vi "Set Channel - GPIO DO.vi"(6 "GPIO Pull":T1, 8 "error in (no error)":errorcluster, 9 "GPIO Number":T2=-1, 10 "Tag":string, 11 "CTI_GPIO_DigitalOut in":refnum<class "CTI_GPIO_DigitalOut.lvclass">) -> (0 "error out":errorcluster, 3 "CTI_GPIO_DigitalOut out":refnum<class "CTI_GPIO_DigitalOut.lvclass">)   [LabVIEW 2021, in "CTI_GPIO_DigitalOut.lvclass"]
uses:
  CTI_GPIO_DigitalOut.lvclass
  <vilib>/CTI/CTI Drivers/CTI/GPIO Number.ctl
  <vilib>/CTI/CTI Drivers/CTI/GPIO Pull.ctl
  <vilib>/CTI/CTI Drivers/CTI/CTI.lvlib
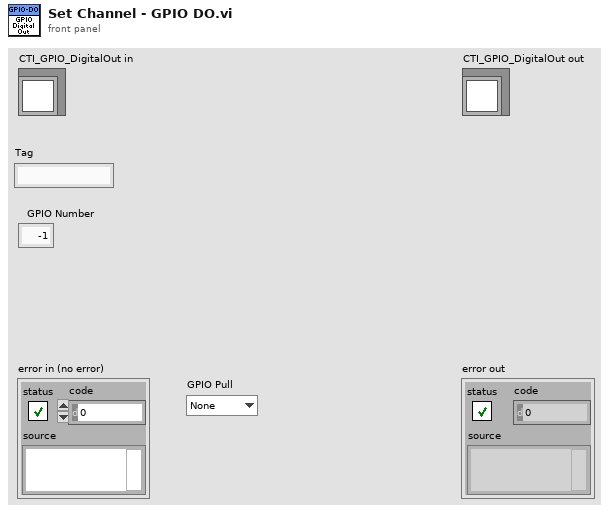
[diagram p1: front panel]
types:
  T1 = typedef "CTI.lvlib/GPIO Pull.ctl" = enum16{"None", "Up", "Down", "Both"}
  T2 = typedef "CTI.lvlib/GPIO Number.ctl" = i8
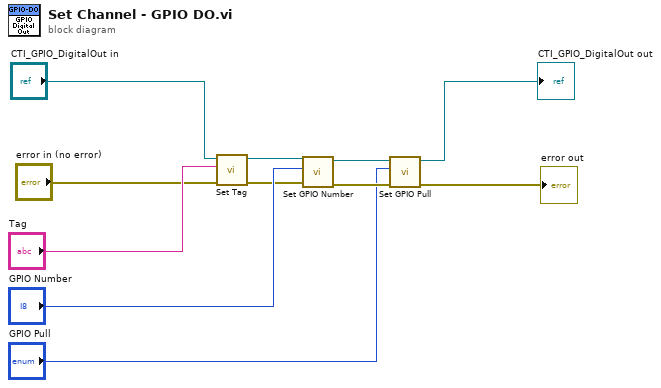
[diagram p0: block diagram]
diagram:
  n1 = call-dynamic "Set Tag.vi"("error in (no error)"="error in (no error)", "Tag"="Tag", "CTI_GPIO_DigitalOut in"="CTI_GPIO_DigitalOut in") -> ("error out"=w7:errorcluster, "CTI_GPIO_DigitalOut out"=w8:refnum<class "CTI_GPIO_DigitalOut.lvclass">)  [unwired: 7 in]
  n2 = call-dynamic "Set GPIO Number.vi"("error in (no error)"=w7, "GPIO Number"="GPIO Number", "CTI_GPIO_DigitalOut in"=w8) -> ("error out"=w5:errorcluster, "CTI_GPIO_DigitalOut out"=w4:refnum<class "CTI_GPIO_DigitalOut.lvclass">)  [unwired: 7 in]
  n3 = call-dynamic "Set GPIO Pull.vi"("error in (no error)"=w5, "GPIO Pull"="GPIO Pull", "CTI_GPIO_DigitalOut in"=w4) -> ("error out"=→"error out":errorcluster, "CTI_GPIO_DigitalOut out"=→"CTI_GPIO_DigitalOut out":refnum<class "CTI_GPIO_DigitalOut.lvclass">)  [unwired: 7 in]
